vi "Clean Error Message.vi"(11 "source":string) -> (3 "message":string)   [LabVIEW 2020, in "MCP Server.lvlib"]
doc: "Returns the human readable part of a LabVIEW error source, so that no markup and no VI call chain reaches an MCP client.\n\nThe result is the text after the <ERR> marker (the whole source if there is none), cut off before the call chain that LabVIEW appends and then cleaned by Strip Error Details.vi (VI call chain, file paths, tags, line breaks)."
uses:
  MCP Server.lvlib
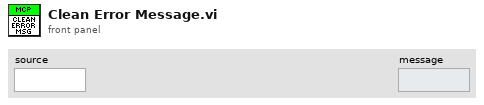
[diagram p1: front panel]
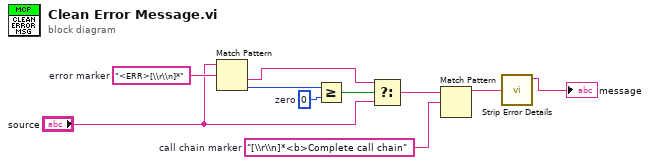
[diagram p0: block diagram]
diagram:
  w3 = "[\\r\\n]*<b>Complete call chain"  # call chain marker
  w8 = 0  # zero
  w10 = "<ERR>[\\r\\n]*"  # error marker
  n1 = Match Pattern(string="source", regular expression=w10) -> (after substring=w7:string, offset past match=w9:i32)  [unwired: 1 in, 2 out]
  n2 = Greater Or Equal?(x=w9, y=w8) -> (x >= y?=w6:bool)
  n3 = Select(t=w7, s=w6, f="source") -> (s? t:f=w4:string)
  n4 = Match Pattern(string=w4, regular expression=w3) -> (before substring=w2:string)  [unwired: 1 in, 3 out]
  n5 = call "Strip Error Details.vi"("text"=w2) -> ("text out"=→"message":string)  [unwired: 9 in, 1 out]
